vi "MaP incremente.vi"() -> ()   [LabVIEW 2020]
panel:
  out "value":dbl
  in  "Cluster_de_depart":T1={"fonction"="incremente", "parameters"={"x"=-2.1235999999999997}}
  out "data string":string
  out "JSON string":string="{\n  \"my_cluster_name\":{\n    \"type\":\"cluster\",\n    \"fields\":{\n      \"my_name\":{\"type\":\"DBL\"},\n      \"my_name2\":{\"type\":\"I32\"},\n      \"my_bool_array\":{\n        \"type\":\"Array\",\n        \"dimensions\":1,\n        \"element\":{\"type\":\"Boolean\"}\n      },\n      \"Array of clusters\":{\n        \"type\":\"Array\",\n        \"dimensions\":2,\n        \"element\":{\n          \"my_cluster_name\":{\n            \"type\":\"cluster\",\n            \"fields\":{\n              \"my_name\":{\"type\":\"DBL\"},\n              \"my_name2\":{\"type\":\"I32\"},\n              \"my_bool_array\":{\n                \"type\":\"Array\",\n                \"dimensions\":1,\n                \"element\":{\"type\":\"Boolean\"}\n              }\n            }\n          }\n        }\n      }\n    }\n  }\n}"
  out "data out (hex)":string
  out "JSON string reçue":string
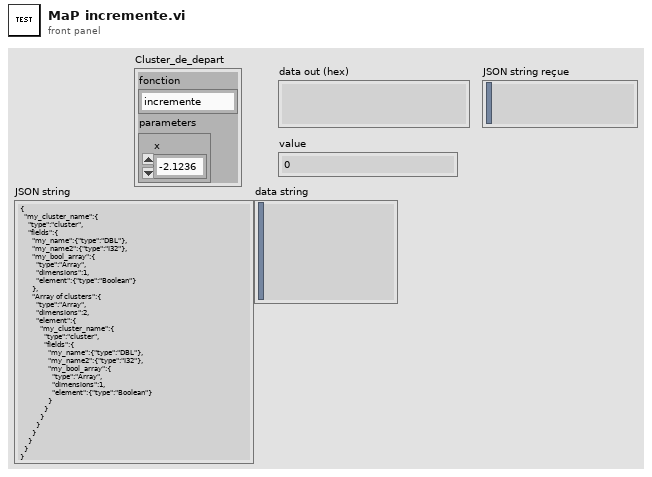
[diagram p1: front panel]
types:
  T1 = cluster{"fonction":string, "parameters":cluster{"x":dbl}}
  T2 = enum16{"big-endian, network order", "native, host order", "little-endian"}
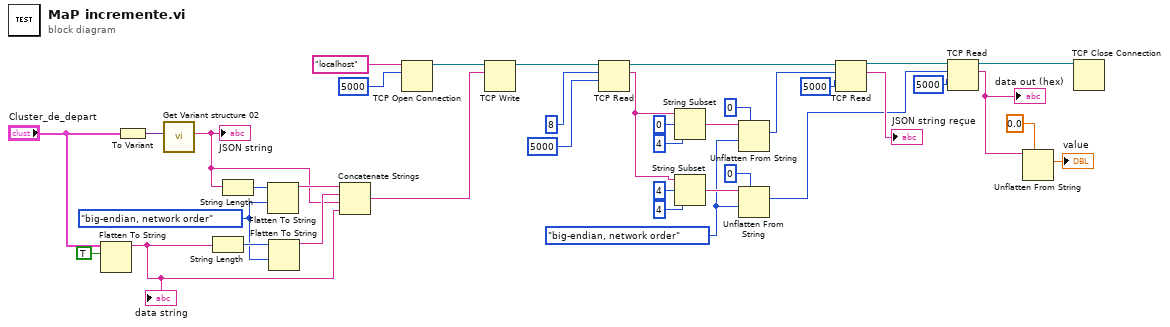
[diagram p0: block diagram]
diagram:
  w9 = T2."big-endian, network order" ("byte order (0:big-endian, network order)")
  w23 = T2."big-endian, network order" ("byte order (0:big-endian, network order)")
  n1 = Flatten To String(anything="Cluster_de_depart", prepend array or string size? (T)=TRUE) -> (data string=w8:string)  [unwired: 2 in, 2 out]
  "data string" <- w8
  n2 = To Variant(anything="Cluster_de_depart") -> (Variant=w5:variant)
  n3 = call "Get Variant structure 02.vi"("variant in"=w5) -> ("<JSON>"=w7:string)  [unwired: 10 in]
  "JSON string" <- w7
  n4 = String Length(string=w8) -> (length=w11:i32)
  n5 = String Length(string=w7) -> (length=w12:i32)
  n6 = Flatten To String(anything=w12, byte order (0:big-endian, network order)=w9) -> (data string=w13:string)  [unwired: 2 in, 2 out]
  n7 = Flatten To String(anything=w11, byte order (0:big-endian, network order)=w9) -> (data string=w10:string)  [unwired: 2 in, 2 out]
  n8 = Concatenate Strings(w13, w10, w7, w8) -> (w4:string)
  n9 = TCP Open Connection(address="localhost", remote port or service name=u16 5000) -> (connection ID=w36:refnum<k5>)  [unwired: 3 in, 1 out]
  n10 = TCP Write(connection ID=w36, data in=w4) -> (connection ID out=w33:refnum<k5>)  [unwired: 2 in, 2 out]
  n11 = TCP Read(connection ID=w33, bytes to read=8, 9:5000 ("timeout ms (25000)")) -> (connection ID out=w21:refnum<k5>, data out=w28:string)  [unwired: 2 in, 1 out]
  n12 = String Subset(string=w28, offset (0)=0, length (rest)=4 ("length (rest)")) -> (substring=w27:string)
  n13 = String Subset(string=w28, offset (0)=4, length (rest)=4 ("length (rest)")) -> (substring=w25:string)
  n14 = Unflatten From String(type=0 ("offset (0)"), binary string=w27, byte order (0:big-endian, network order)=w23) -> (value=w20:i32)  [unwired: 2 in, 2 out]
  n15 = Unflatten From String(type=0 ("offset (0)"), binary string=w25, byte order (0:big-endian, network order)=w23) -> (value=w15:i32)  [unwired: 2 in, 2 out]
  n16 = TCP Read(connection ID=w21, bytes to read=w20, 9:5000 ("timeout ms (25000)")) -> (connection ID out=w17:refnum<k5>, data out=→"JSON string reçue":string)  [unwired: 2 in, 1 out]
  n17 = TCP Read(connection ID=w17, bytes to read=w15, 9:5000 ("timeout ms (25000)")) -> (connection ID out=w16:refnum<k5>, data out=w1:string)  [unwired: 2 in, 1 out]
  "data out (hex)" <- w1
  n18 = Unflatten From String(type=0.0, binary string=w1) -> (value=→"value":dbl)  [unwired: 3 in, 2 out]
  n19 = TCP Close Connection(connection ID=w16) -> ()  [unwired: 2 in, 2 out]
